vi "IMU Get Yaw.vi"   [LabVIEW 2023, in "MrcLib.lvlib"]
doc: "Return the computed Yaw of the built-in sensor. Be sure to select the version that matches the robot controller orientation."
uses:
  <vilib>/MRC/MrcLib.lvlib
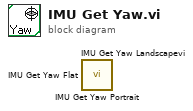
[diagram p0: block diagram]
diagram:
  n1 = call <vilib>:"IMU Get Yaw Portrait.vi"() -> ()  [unwired: 9 in, 3 out]
  n2 = call <vilib>:"IMU Get Yaw Landscapevi.vi"() -> ()  [unwired: 9 in, 3 out]
  n3 = call <vilib>:"IMU Get Yaw Flat.vi"() -> ()  [unwired: 9 in, 3 out]
